vi "setUp.vi"(8 "error in (no error)":errorcluster, 11 "Unit Tests for Runner in":refnum<class "Unit Tests for Runner.lvclass">) -> (0 "error out":errorcluster, 3 "Unit Tests for Runner out":refnum<class "Unit Tests for Runner.lvclass">)   [LabVIEW 2020, in "Unit Tests for Runner.lvclass"]
uses:
  Unit Tests for Runner.lvclass
  C:/projects/caraya/src/classes/Test Runner/Test Runner.lvclass
  Unit Tests for Runner.lvclass/Unit Tests for Runner.ctl
  classes/Test Runner/Test Runner.lvclass
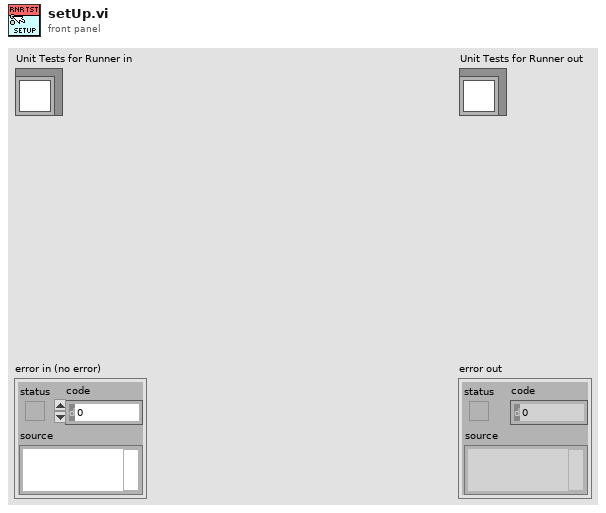
[diagram p1: front panel]
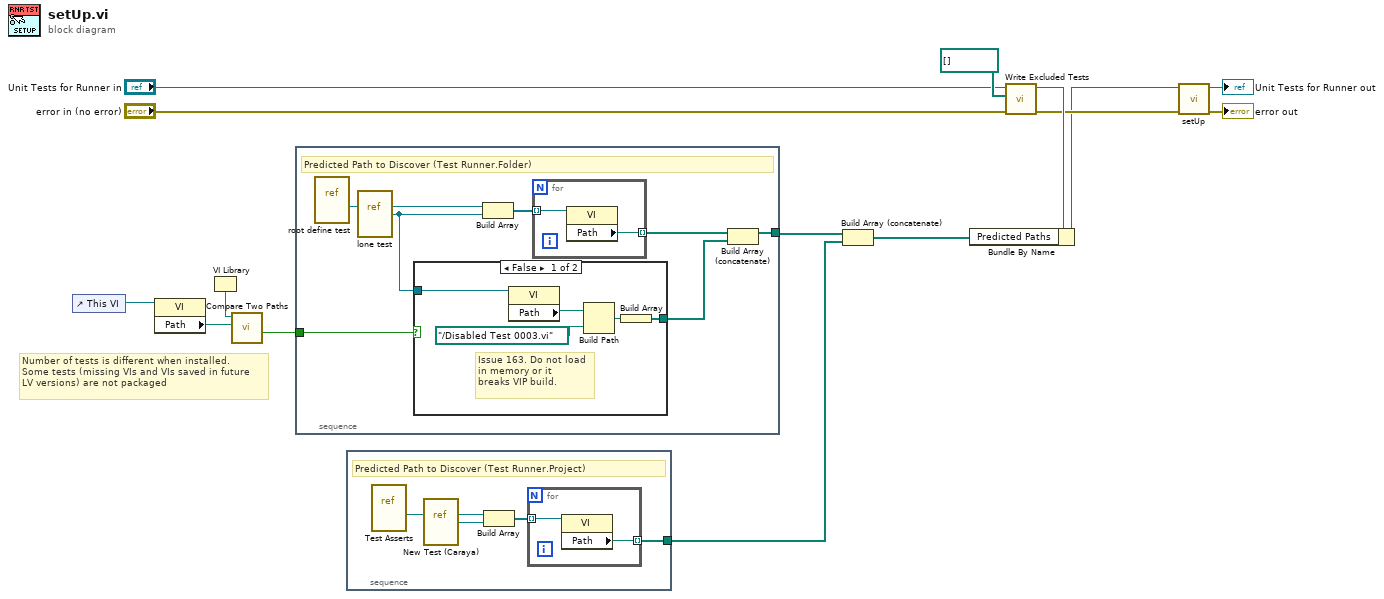
[diagram p0: block diagram]
diagram:
  # "Number of tests is different when installed.\nSome tests (missing VIs and VIs saved in future\nLV versions) are not packaged"
  n1 = control-ref of="This VI"() -> (w4:refnum<vi>)
  n2 = property on="Property Node" class="VI"(reference=w4) -> ("Path"=w3:path)  [unwired: 1 in, 2 out]
  n3 = VI Library() -> (path=w2:path)
  n4 = call <vilib>:"Compare Two Paths.vi"("Path 2"=w3, "Path 1"=w2) -> ("Path 2 Relative to Path 1?"=w1:bool)  [unwired: 6 in, 3 out]
  n5 = stacked-sequence {
    tunnel: [w19] -> w10
    tunnel: w1 -> [w16]
    frame #0 {
      # "Predicted Path to Discover (Test Runner.Folder)"
      n6 = vi-ref "root define test.vi"() -> (w22:refnum<vi>)
      n7 = vi-ref "lone test.vi"() -> (w20:refnum<vi>)
      n8 = case shown="False" w16 {
        tunnel: w20 -> [w27 _]
        tunnel: [w23 _] -> w17
        frame False {
          # "Issue 163. Do not load\nin memory or it\nbreaks VIP build."
          n9 = property on="Property Node" class="VI"(reference=w27) -> ("Path"=w26:path)  [unwired: 1 in, 2 out]
          n10 = Build Path(base path=w26, name or relative path=path "../Disabled Test 0003.vi" ("VI Path")) -> (appended path=w24:path)
          n11 = Build Array(w24) -> (w23:path[])
        }
        frame True {
        }
      }
      n12 = Build Array(w22, w20) -> (w21:refnum<vi>[])
      n13 = for {
        tunnel: w21 -> [w29] mode=indexing
        tunnel: [w28] -> w18 mode=indexing
        n14 = property on="Property Node" class="VI"(reference=w29) -> ("Path"=w28:path)  [unwired: 1 in, 2 out]
      }
      n15 = Build Array (concatenate)(w18, w17) -> (w19:path[])
    }
  }
  n16 = stacked-sequence {
    tunnel: [w31] -> w9
    frame #0 {
      # "Predicted Path to Discover (Test Runner.Project)"
      n17 = vi-ref "Test Asserts.vi"() -> (w33:refnum<vi>)
      n18 = vi-ref "New Test (Caraya).vi"() -> (w30:refnum<vi>)
      n19 = Build Array(w33, w30) -> (w32:refnum<vi>[])
      n20 = for {
        tunnel: w32 -> [w35] mode=indexing
        tunnel: [w34] -> w31 mode=indexing
        n21 = property on="Property Node" class="VI"(reference=w35) -> ("Path"=w34:path)  [unwired: 1 in, 2 out]
      }
    }
  }
  n22 = Build Array (concatenate)(w10, w9) -> (w8:path[])
  n23 = call "Write Excluded Tests.vi"("error in (no error)"="error in (no error)", "Excluded Tests"=path[] [], "Test Runner in"="Unit Tests for Runner in") -> ("error out"=w7:errorcluster, "Test Runner out"=w12:refnum<class "Unit Tests for Runner.lvclass">)  [unwired: 7 in]
  n24 = Bundle By Name(cluster=w12, "Predicted Paths"=w8) -> (w6:refnum<class "Unit Tests for Runner.lvclass">)
  n25 = call-parent "setUp.vi"("error in (no error)"=w7, "Test Runner in"=w6) -> ("error out"=→"error out":errorcluster, "Test Runner out"=→"Unit Tests for Runner out":refnum<class "Unit Tests for Runner.lvclass">)  [unwired: 8 in]
